vi "libssh2_agent_list_identities.vi"(8 "error in (no error)":errorcluster, 11 "agent":T1) -> (0 "error out":errorcluster)   [LabVIEW 2017, in "libssh2.lvlib"]
doc: "Request a list of public keys from the SSH agent. Call <B>libssh2_agent_get_identity</B> to get a public key."
uses:
  libssh2.lvlib
  Agent Refnum.ctl
  Acquire Session.vi
  Release Session.vi
  Not An Agent.vi
  <vilib>/Utility/error.llb/Error Cluster From Error Code.vi
  Global Settings.vi
  Read Agent Refnum.vi
  Read Session Refnum.vi
  <vilib>/Utility/semaphor.llb/Acquire Semaphore.vi
  <vilib>/Utility/semaphor.llb/Release Semaphore.vi
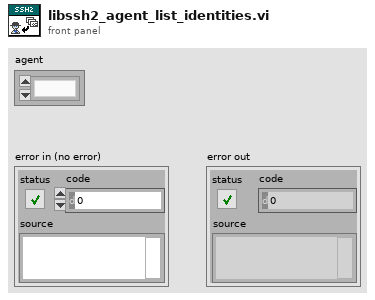
[diagram p1: front panel]
types:
  T1 = typedef "libssh2.lvlib/Agent Refnum.ctl" = refnum<k1>
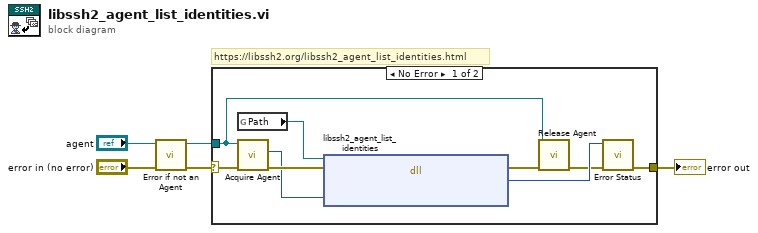
[diagram p0: block diagram]
diagram:
  # "https://libssh2.org/libssh2_agent_list_identities.html"
  n1 = call "Error if not an Agent.vi"("error in (no error)"="error in (no error)", "agent"="agent") -> ("error out"=w3:errorcluster, "agent out"=w2:T1)  [unwired: 8 in]
  n2 = case shown="No Error" w3 {
    selector: w3 -> [w13 w15]
    tunnel: [w14 w15] -> w5
    tunnel: w2 -> [w6 _]
    frame No Error {
      n3 = global read "Global Settings.vi" "Path"() -> (w10:path)
      n4 = call "Acquire Agent.vi"("error in (no error)"=w13, "agent"=w6) -> ("error out"=w9:errorcluster, "LIBSSH2_AGENT*"=w8:u64)  [unwired: 8 in]
      n5 = dll-call lib="?" fn="libssh2_agent_list_identities"(path in=w10, error in=w9, "agent"=w8) -> (error out=w11:errorcluster, "return value"=w12:i32)  [unwired: 2 in, 1 out]
      n6 = call "Release Agent.vi"("error in (no error)"=w11, "agent"=w6) -> ("error out"=w7:errorcluster)  [unwired: 9 in]
      n7 = call "Error Status.vi"("error in (no error)"=w7, "return value"=w12) -> ("error out"=w14:errorcluster)  [unwired: 8 in, 1 out]
    }
    frame Error {
    }
  }
  "error out" <- w5
